vi "lvmcp_propconfig.vi"() -> ()   [LabVIEW 2026]
panel:
  out "reference out":refnum<vi>
  out "error out":errorcluster
  out "Set Properties[] (Allow Private)":refnum<vi>[](array[refnum])
  in  "Allow Alternate Names? (F)":bool
  in  "ID Strings[]":string[](array[string])
  in  "Property Node Class Name":string
  in  "reference":refnum<vi>
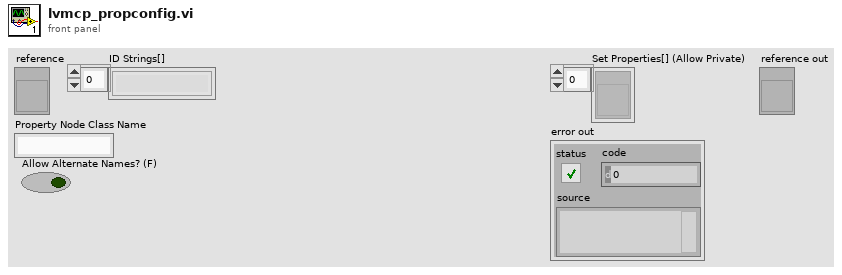
[diagram p1: front panel]
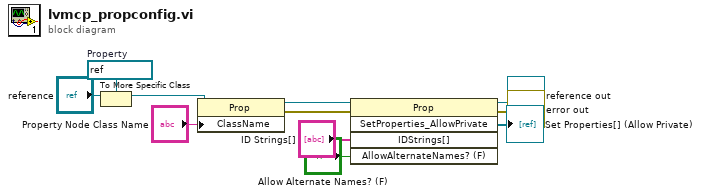
[diagram p0: block diagram]
diagram:
  w11 = refnum<vi> refnum  # Property
  n1 = To More Specific Class(target class=w11, reference="reference") -> (specific class reference=w9:refnum<vi>)  [unwired: 1 in, 1 out]
  n2 = property class="Prop"(reference=w9, "ClassName"="Property Node Class Name") -> (reference out=w7:refnum<vi>, error out=w6:errorcluster)  [unwired: 1 in]
  n3 = invoke class="Prop" method="SetProperties_AllowPrivate"(reference=w7, error in=w6, "IDStrings[]"="ID Strings[]", "AllowAlternateNames? (F)"="Allow Alternate Names? (F)") -> (reference out=→"reference out":refnum<vi>, error out=→"error out":errorcluster, "SetProperties_AllowPrivate"=→"Set Properties[] (Allow Private)":refnum<vi>[])  [unwired: 1 in, 2 out]
